vi "modbus initialize API object.vi"(8 "error in":errorcluster, 11 "Modbus Slave configuration in":refnum<class "Modbus Module configuration.lvclass">) -> (0 "error out":errorcluster, 2 "Clients Count DVR":refnum<data-value>, 3 "Modbus Slave out":refnum<class "Modbus API.lvclass">)   [LabVIEW 2015, in "Modbus Module runtime.lvclass"]
uses:
  Modbus Module runtime.lvclass
  configuration/Modbus Module configuration.lvclass
  <vilib>/NI/Modbus Library/API/Modbus API.lvclass
  configuration/Modbus Module configuration.lvclass/Modbus Module configuration.ctl
  <vilib>/NI/Modbus Library/API/Master/Modbus Master.lvclass
  configuration/Read port (502).vi
  configuration/Read IP address.vi
  configuration/Read serial type.vi
  configuration/Read unit ID.vi
  configuration/Read baud rate.vi
  configuration/Read VISA resource name.vi
  configuration/Read parity (even).vi
  configuration/Read flow control (none).vi
  configuration/Read class.vi
  <vilib>/NI/Modbus Library/API/Wrapper/Create TCP Slave.vi
  <vilib>/NI/Modbus Library/API/Wrapper/Create TCP Master.vi
  configuration/get wire mode.vi
  configuration/read force wire mode.vi
  <vilib>/NI/Modbus Library/API/Wrapper/Create Serial Master.vi
  <vilib>/NI/Modbus Library/API/Wrapper/Create Serial Slave.vi
  <vilib>/NI/Modbus Library/API/Wrapper/API Main.lvlib
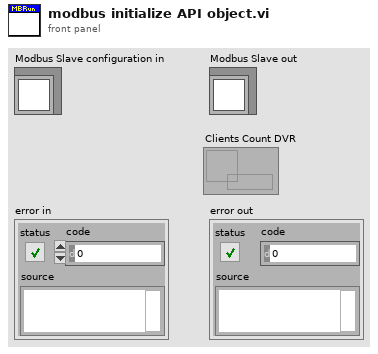
[diagram p1: front panel]
types:
  T1 = typedef "Modbus Slave configuration.lvclass/modbus class.ctl" = enum16{"TCP master", "TCP slave", "serial master", "serial slave"}
  T2 = cluster{"serial master instance":refnum<class "Modbus Master.lvclass">, "Clients Count DVR":refnum<data-value>}
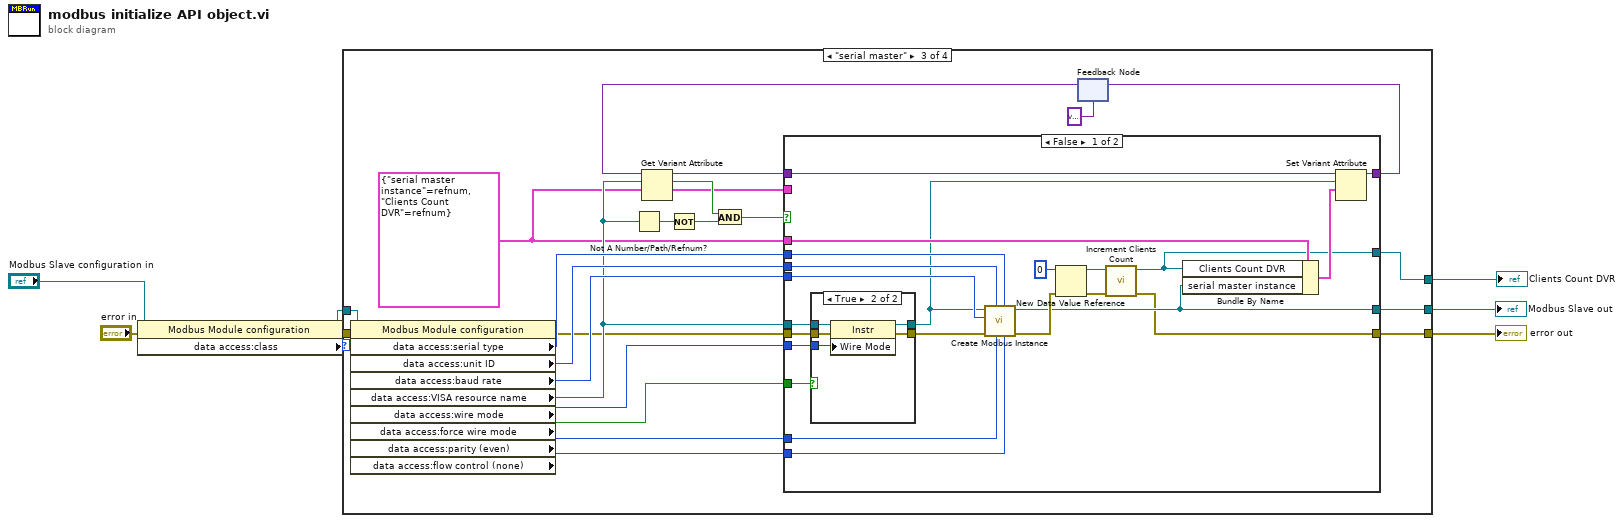
[diagram p0: block diagram]
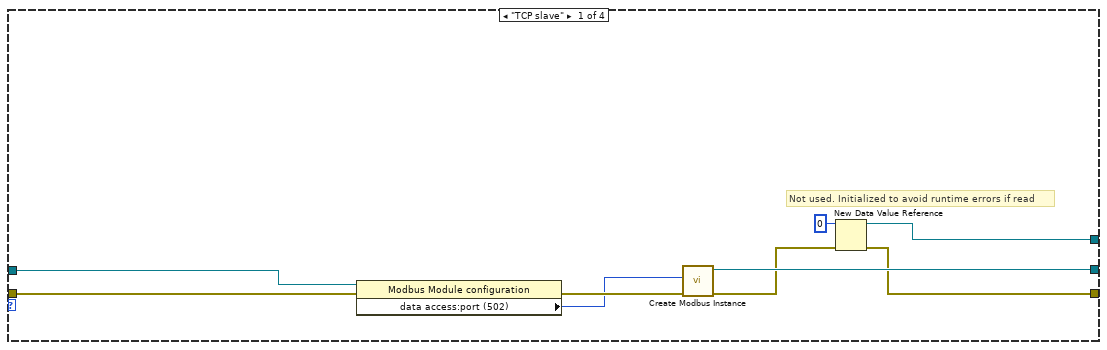
[diagram p2: hidden frame]
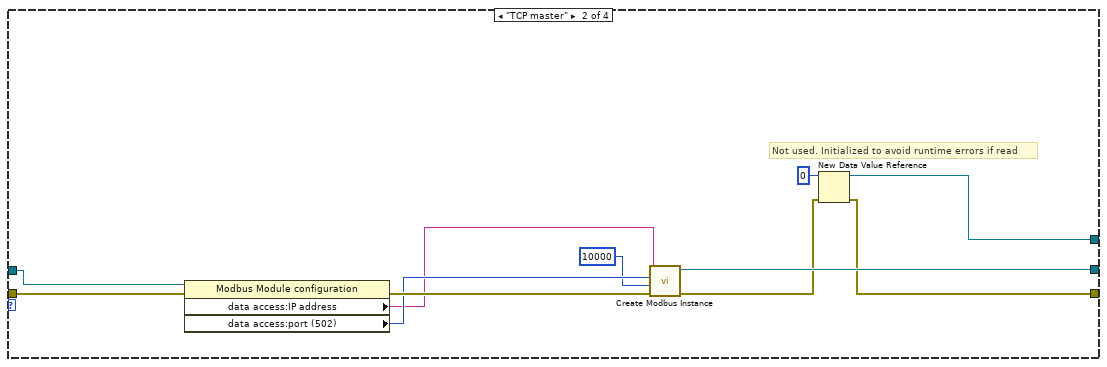
[diagram p3: hidden frame]
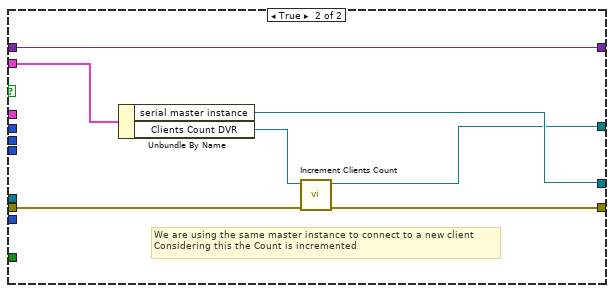
[diagram p5: hidden frame]
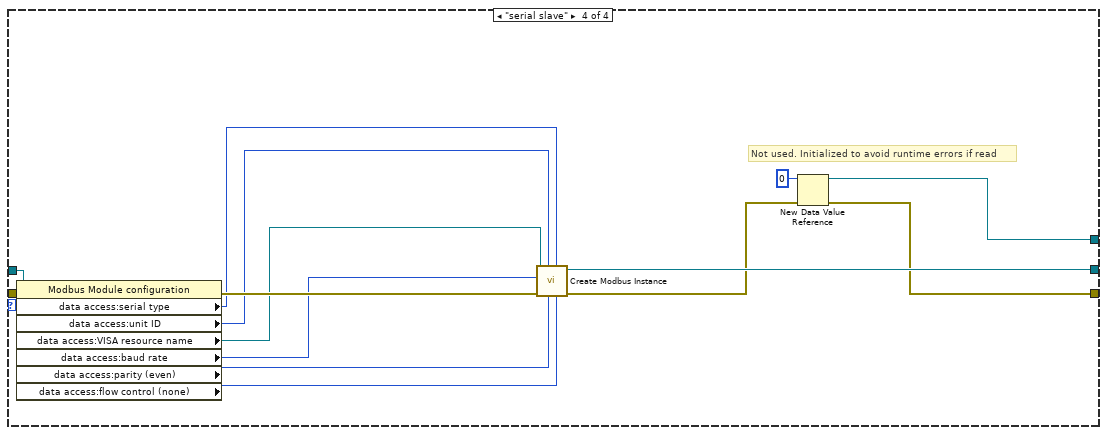
[diagram p6: hidden frame]
diagram:
  n1 = property class="Modbus Module configuration"(reference="Modbus Slave configuration in", error in="error in") -> (reference out=w2:refnum<class "Modbus Module configuration.lvclass">, error out=w5:errorcluster, "data access:class"=w3:T1)
  n2 = case shown="\"serial master\"" w3 {
    tunnel: [w9 w19 w31 w89] -> w8
    tunnel: [w17 w28 w52 w102] -> w6
    tunnel: w5 -> [w16 w27 w51 w101]
    tunnel: w2 -> [w14 w25 w50 w99]
    tunnel: [w11 w20 w29 w91] -> w1
    frame "TCP slave" {
      # "Not used. Initialized to avoid runtime errors if read"
      n3 = property class="Modbus Module configuration"(reference=w14, error in=w16) -> (error out=w15:errorcluster, "data access:port (502)"=w13:u16)  [unwired: 1 out]
      n4 = call-poly <vilib>:"Create Modbus Instance.vi"("error in"=w15, "port (502)"=w13) -> ("error out"=w10:errorcluster, "TCP slave instance"=w17:refnum<class "Modbus Slave.lvclass">)  [unwired: 8 in]
      n5 = New Data Value Reference(data value=0, error in=w10) -> (data value reference=w11:refnum<data-value>, error out=w9:errorcluster)
    }
    frame "TCP master" {
      # "Not used. Initialized to avoid runtime errors if read"
      n6 = property class="Modbus Module configuration"(reference=w25, error in=w27) -> (error out=w26:errorcluster, "data access:IP address"=w22:string, "data access:port (502)"=w24:u16)  [unwired: 1 out]
      n7 = call-poly <vilib>:"Create Modbus Instance.vi"("error in"=w26, "connect timeout ms"=10000, "port (502)"=w24, "address"=w22) -> ("error out"=w18:errorcluster, "TCP master instance"=w28:refnum<class "Modbus Master.lvclass">)  [unwired: 6 in]
      n8 = New Data Value Reference(data value=0, error in=w18) -> (data value reference=w20:refnum<data-value>, error out=w19:errorcluster)
    }
    frame "serial master" {
      w33 = T2 {"serial master instance"=refnum, "Clients Count DVR"=refnum}
      n9 = property class="Modbus Module configuration"(reference=w50, error in=w51) -> (error out=w30:errorcluster, "data access:serial type"=w49:enum16{"RTU", "ASCII"}, "data access:unit ID"=w48:u8, "data access:baud rate"=w47:u32, "data access:VISA resource name"=w37:refnum<visa-resource-name>, "data access:wire mode"=w46:i16, "data access:force wire mode"=w45:bool, "data access:parity (even)"=w44:u16, "data access:flow control (none)"=w43:u16)  [unwired: 1 out]
      n10 = Not A Number/Path/Refnum?(number/path/refnum=w37) -> (NaN/Path/Refnum?=w39:bool)
      n11 = Not(x=w39) -> (.not. x?=w38:bool)
      n12 = feedback #1(variant) -> (w41:variant)
      n13 = Get Variant Attribute(Variant=w41, name=w37, default value (empty Variant)=w33) -> (duplicate Variant=w32:variant, found=w36:bool, value=w34:T2)  [unwired: 1 in, 1 out]
      n14 = And(x=w36, y=w38) -> (x .and. y?=w35:bool)
      n15 = case shown="False" w35 {
        tunnel: [w61 w86] -> w52
        tunnel: [w73 w88] -> w40
        tunnel: w49 -> [w72 _]
        tunnel: w48 -> [w71 _]
        tunnel: w47 -> [w70 _]
        tunnel: w37 -> [w69 _]
        tunnel: w46 -> [w68 _]
        tunnel: w45 -> [w67 _]
        tunnel: w44 -> [w66 _]
        tunnel: w43 -> [w65 _]
        tunnel: w33 -> [w62 _]
        tunnel: w34 -> [_ w87]
        tunnel: w32 -> [w59 w88]
        tunnel: [w55 w83] -> w31
        tunnel: w30 -> [w54 w84]
        tunnel: [w53 w82] -> w29
        frame False {
          n16 = case shown="True" w67 {
            tunnel: [w75 w81] -> w74
            tunnel: [w76 w80] -> w58
            tunnel: w69 -> [w76 w79]
            tunnel: w68 -> [_ w78]
            tunnel: w54 -> [w75 w77]
            frame False {
            }
            frame True {
              n17 = property class="Instr"(reference=w79, error in=w77, "Wire Mode"=w78) -> (reference out=w80:refnum<visa-resource-name>, error out=w81:errorcluster)
            }
          }
          n18 = call-poly <vilib>:"Create Modbus Instance.vi"("flow control (none)"=w65, "serial type"=w72, "parity (even)"=w66, "unit ID"=w71, "error in"=w74, "baud rate"=w70, "VISA resource name"=w58) -> ("error out"=w64:errorcluster, "serial master instance"=w61:refnum<class "Modbus Master.lvclass">)  [unwired: 3 in]
          n19 = New Data Value Reference(data value=0, error in=w64) -> (data value reference=w57:refnum<data-value>, error out=w56:errorcluster)
          n20 = call "Increment Clients Count.vi"("error in (no error)"=w56, "Data Value Reference in"=w57) -> ("error out"=w55:errorcluster, "Data Value Reference out"=w53:refnum<data-value>)  [unwired: 7 in, 1 out]
          n21 = Bundle By Name(cluster=w62, "Clients Count DVR"=w53, "serial master instance"=w61) -> (w60:T2)
          n22 = Set Variant Attribute(Variant=w59, name=w58, value=w60) -> (Variant out=w73:variant)  [unwired: 1 in, 2 out]
        }
        frame True {
          # "We are using the same master instance to connect to a new client\nConsidering this the Count is incremented"
          n23 = Unbundle By Name(w87) -> ("serial master instance"=w86:refnum<class "Modbus Master.lvclass">, "Clients Count DVR"=w85:refnum<data-value>)
          n24 = call "Increment Clients Count.vi"("error in (no error)"=w84, "Data Value Reference in"=w85) -> ("error out"=w83:errorcluster, "Data Value Reference out"=w82:refnum<data-value>)  [unwired: 7 in, 1 out]
        }
      }
      n25 = feedback-in #1(w40) -> ()
    }
    frame "serial slave" {
      # "Not used. Initialized to avoid runtime errors if read"
      n26 = property class="Modbus Module configuration"(reference=w99, error in=w101) -> (error out=w100:errorcluster, "data access:serial type"=w96:enum16{"RTU", "ASCII"}, "data access:unit ID"=w95:u8, "data access:VISA resource name"=w94:refnum<visa-resource-name>, "data access:baud rate"=w93:u32, "data access:parity (even)"=w98:u16, "data access:flow control (none)"=w97:u16)  [unwired: 1 out]
      n27 = call-poly <vilib>:"Create Modbus Instance.vi"("flow control"=w97, "serial type"=w96, "parity (even)"=w98, "unit ID"=w95, "error in"=w100, "baud rate (9600)"=w93, "VISA resource name"=w94) -> ("error out"=w90:errorcluster, "serial slave instance"=w102:refnum<class "Modbus Slave.lvclass">)  [unwired: 3 in]
      n28 = New Data Value Reference(data value=0, error in=w90) -> (data value reference=w91:refnum<data-value>, error out=w89:errorcluster)
    }
  }
  "error out" <- w8
  "Modbus Slave out" <- w6
  "Clients Count DVR" <- w1
